vi "Host_Validate_Config.vi"(8 "error in (no error)":errorcluster={"status"=FALSE, "code"=0, "source"="\"\""}, 11 "Editable config package":string) -> (0 "error out":errorcluster={"status"=FALSE, "code"=0, "source"="\"\""}, 2 "status ok":bool, 3 "Diagnostics list":string)   [LabVIEW 2026]
doc: "INTENT: Run initial editing checks. LOGIC: Call structural, semantic and plugin validation locally before publish; show precise path to failures."
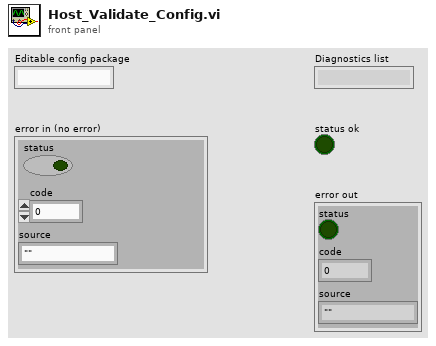
[diagram p1: front panel]
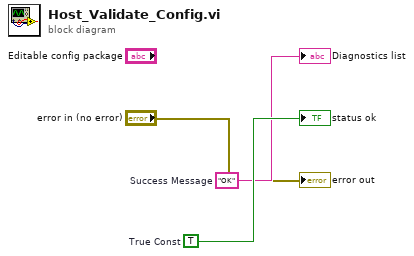
[diagram p0: block diagram]
diagram:
  w3 = TRUE  # True Const
  w2 = "OK"  # Success Message
  "Diagnostics list" <- w2
  "status ok" <- w3
  "error out" <- "error in (no error)"
